vi "Rollover Events.vi"() -> ()   [LabVIEW 2018]
uses:
  src/api/logger_class/Log Levels.ctl
  bc269cd9-d162-4013-a312-bd866d79ee19.vi
  src/api/configuration/handlers/file_handler/File Handler.lvclass
  C:/Users/Colin/Documents/software_projects/labview/glog/src/api/extension/formatting_handler_interface/Formatting Handler.lvclass
  src/api/logger_class/Log (Parts).vi
  src/api/logger_class/Logger.lvclass
panel:
  in  "Stop":bool
  out "Source":string
  out "Current Log File":path
  out "sources":string[](array[string])
  out "log files":path[](array[path])
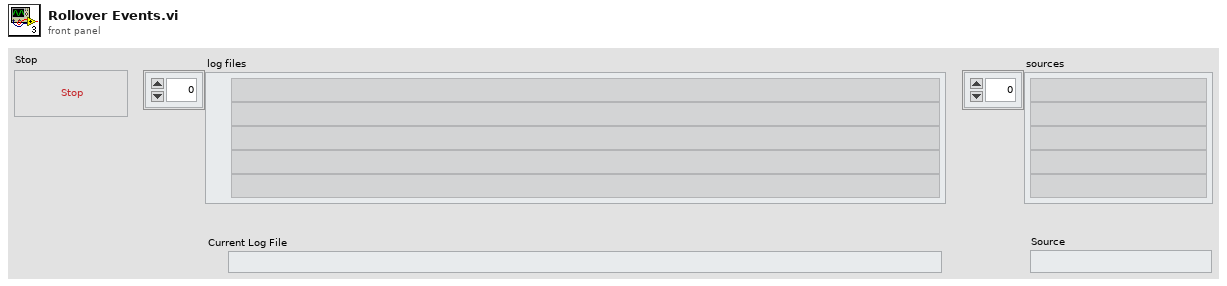
[diagram p1: front panel]
types:
  T1 = typedef "GLog.lvlib/File Handler.lvclass/Events.ctl" = cluster{"File Rollover":refnum<user-event>}
  T2 = typedef "GLog.lvlib/Logger.lvclass/Log Levels.ctl" = enum16{"Trace", "Debug", "Info", "Warning", "Error", "Critical"}
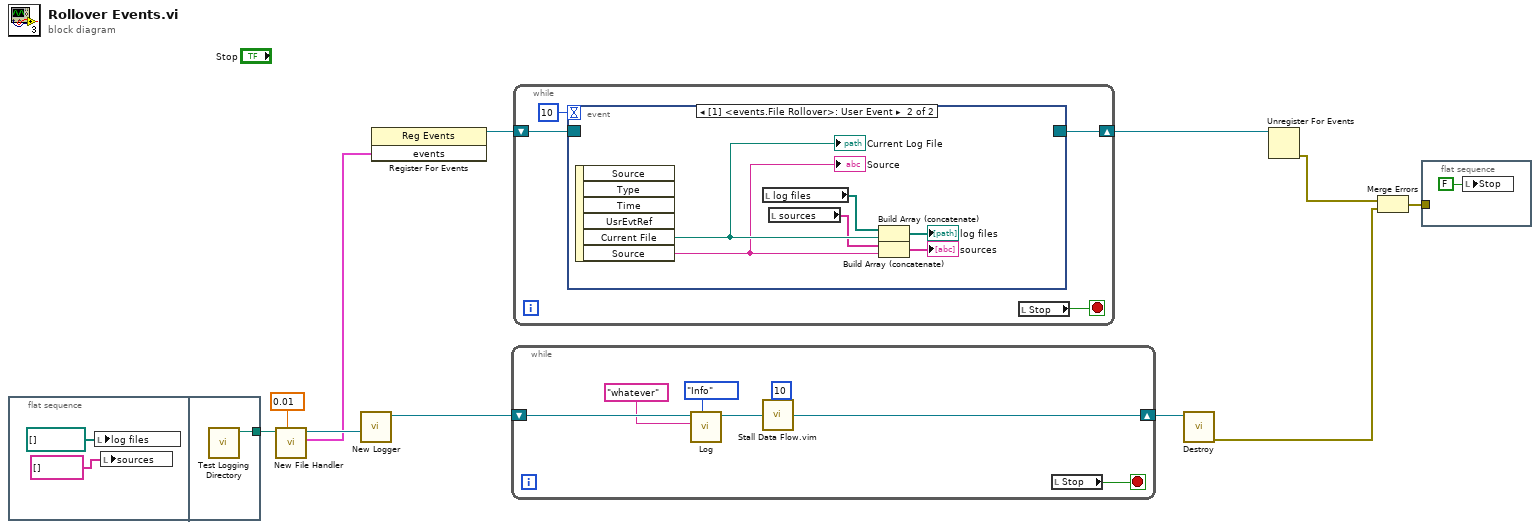
[diagram p0: block diagram]
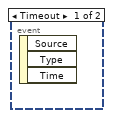
[diagram p2: hidden frame]
diagram:
  n1 = flat-sequence {
    tunnel: [w14] -> w1
    frame #0 {
      n2 = local write "log files"(path[] [] ("log files")) -> ()
      n3 = local write "sources"(string[] [] ("sources")) -> ()
    }
    frame #1 {
      n4 = call "Test Logging Directory.vi"() -> ("test logging directory"=w14:path)  [unwired: 11 in]
    }
  }
  n5 = call "New File Handler.vi"("max file size [MB](50)"=0.01, "log directory (<app dir>/logs)"=w1) -> ("events"=w9:T1, "file handler"=w11:refnum<class "File Handler.lvclass">)  [unwired: 7 in, 1 out]
  n6 = call "New Logger.vi"("log handler (file handler)"=w11) -> ("logger"=w7:refnum<class "Logger.lvclass">)  [unwired: 9 in, 1 out]
  n7 = register-events(w9) -> (reference out=w8:refnum<event-registration>)  [unwired: 2 in, 1 out]
  n8 = while {
    shift-right: [w18] -> w6
    shift-left: w7 -> [w21]
    stop <- w16 stop-if-true
    n9 = call-poly "Log.vi"("log level"=Log_Levels."Info", "message"="whatever", "logger in"=w21) -> ("logger out"=w19:refnum<class "Logger.lvclass">)  [unwired: 8 in]
    n10 = call "Stall Data Flow.vim"("value in"=w19, "milliseconds to wait"=u32 10) -> ("value out"=w18:refnum<class "Logger.lvclass">)  [unwired: 1 out]
    n11 = local read "Stop"() -> (w16:bool)
  }
  n12 = while {
    shift-right: [w24] -> w5
    shift-left: w8 -> [w25]
    stop <- w23 stop-if-true
    n13 = event shown="[1] <events.File Rollover>: User Event" {
      selector: w25 -> [_ _]
      dyn-events: [_ _] -> w24
      timeout: 10 -> [_ _]
      event Timeout {
        n14 = event-data() -> ()  [unwired: 1 in, 3 out]
      }
      event User Event {
        n15 = event-data() -> ("Current File"=w31:path, "Source"=w30:string)  [unwired: 1 in, 4 out]
        "Current Log File" <- w31
        "Source" <- w30
        n16 = local read "log files"() -> (w27:path[])
        n17 = local read "sources"() -> (w26:string[])
        n18 = Build Array (concatenate)(w27, w31) -> (→"log files":path[])
        n19 = Build Array (concatenate)(w26, w30) -> (→"sources":string[])
      }
    }
    n20 = local read "Stop"() -> (w23:bool)
  }
  n21 = call "Destroy.vi"("logger in"=w6) -> ("error out"=w3:errorcluster)  [unwired: 9 in, 1 out]
  n22 = Unregister For Events(event registration refnum=w5) -> (error out=w4:errorcluster)  [unwired: 1 in]
  n23 = Merge Errors(w4, w3) -> (w2:errorcluster)
  n24 = flat-sequence {
    tunnel: w2 -> [_]
    frame #0 {
      n25 = local write "Stop"(FALSE ("Stop")) -> ()
    }
  }
